vi "UE_Operating_Point_Ready.vi"(3 "mode_valid":bool, 4 "flow_achieved":bool, 5 "pressure_achieved":bool) -> (2 "ready":bool)   [LabVIEW 2026]
doc: "INTENT: Combine pressure, flow and mode validity for a combined VTU point. INPUTS: pressure_achieved (bool), flow_achieved (bool), mode_valid (bool). OUTPUTS: ready (bool). DESIGN CONSTRAINT: Not a substitute for individual controller status or stale-signal checks. REQUIREMENTS: SRS-F-019. No physical hardware side effects. Acceptance requires native LabVIEW compilation and behavioral testing."
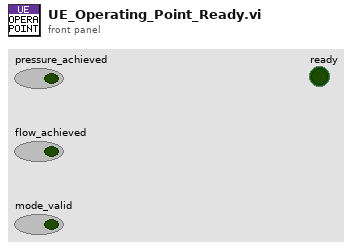
[diagram p1: front panel]
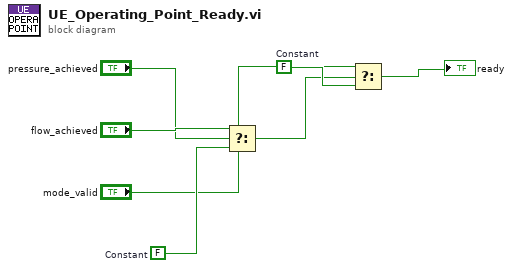
[diagram p0: block diagram]
diagram:
  w6 = FALSE  # Constant
  w4 = FALSE  # Constant
  n1 = Select(t="flow_achieved", s="pressure_achieved", f=w4) -> (s? t:f=w5:bool)
  n2 = Select(t="mode_valid", s=w5, f=w6) -> (s? t:f=→"ready":bool)
